vi "mupSetExpr.vi"(8 "error in (no error)":errorcluster, 10 "szExpr":string, 11 "muPar in":u64) -> (0 "error out":errorcluster, 3 "muPar out":u64)   [LabVIEW 2018, in "mupLib.lvlib"]
doc: "Set the expression string. Multiple expressions can be input using comma as delimiter."
uses:
  mupLib.lvlib
  libmuparser-lv.dll
panel:
  # "Set the expression string. Multiple expressions can be input using comma as delimiter."
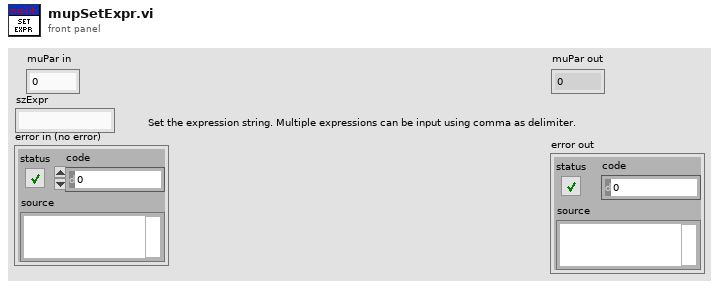
[diagram p1: front panel]
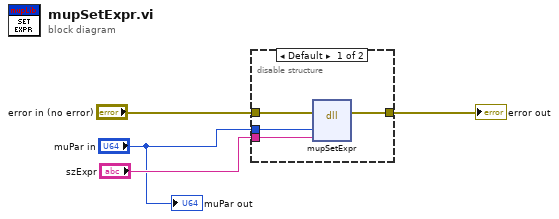
[diagram p0: block diagram]
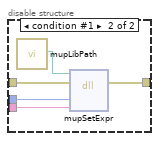
[diagram p2: hidden frame]
diagram:
  n1 = disable-structure shown="Default" {
    disable-tunnel: "szExpr" -> [w8 w13]
    disable-tunnel: "error in (no error)" -> [w7 w12]
    disable-tunnel: [w6 w11] -> w2
    disable-tunnel: "muPar in" -> [w5 w10]
    frame condition #0 (active) {
      n2 = dll-call lib="C:/Users/leonidas/Documents/GitHub/LV-muParser/mupLib/libmuparser-lv.dll" fn="mupSetExpr"(error in=w7, "hParser"=w5, "szExpr"=w8) -> (error out=w6:errorcluster)  [unwired: 5 in, 1 out]
    }
    frame condition #1 {
      n3 = call "mupLibPath.vi"() -> ("libmuparser path"=w9:path)  [unwired: 11 in]
      n4 = dll-call lib="C:/Users/leonidas/Documents/GitHub/LV-muParser/mupLib/libmuparser-lv.dll" fn="mupSetExpr"(path in=w9, error in=w12, "hParser"=w10, "szExpr"=w13) -> (error out=w11:errorcluster)  [unwired: 4 in, 1 out]
    }
  }
  "error out" <- w2
  "muPar out" <- "muPar in"
